vi "Test Launcher API.vi"() -> ()   [LabVIEW 2026]
doc: "Launcher API Tester."
uses:
  Mode.ctl
  ReplayMode.ctl
  RecordMode.ctl
  <vilib>/Utility/error.llb/DialogType.ctl
  Capture detection loop data--cluster.ctl
  663af669-4b40-4be5-87dd-68c6d9059199.vi
  <vilib>/Utility/error.llb/Search and Replace Pattern (string).vi
  <vilib>/JDP Science/JSONtext/Variant to JSON Text.vi
  <vilib>/JDP Science/JSONtext/LVClass Serializer/JSONtext LVClass Serializer.lvclass
  Launcher.lvlib
  replay/Replay/src/Libraries/Replay/Replay.lvlib
panel:
  in  "Load From Program Data":bool
  in  "key mode":enum16{"RELATIVE", "ABSOLUTE"}(ring)=enum."ABSOLUTE"
  in  "Load User Events":bool
  in  "Multicolumn Listbox":i32(listbox)
  in  "Run ID Replay":string="run-1791981803196"
  in  "Mode":T1={"Replay"=enum."None", "Record"=enum."User Events and Benchmarks"}
  out "last error":errorcluster
  in  "Show Diagram on Init":bool
  in  "Show Block Diagram":bool
  in  "Stop Module":bool
  in  "Start Module":bool
  in  "Hide Module Panel":bool
  in  "Show Module Panel":bool
  out "Status":string
  out "Module Running?":bool
  # "This VI tests the API for the Module."
  # "Set the folder where the runs are located\n\nCreate a loop or launch an asynchronous launcher that detects new runs\nOnce a new run is detected, launches the core module that polls the JSON files of the new run\nOnce the first frame is detected, cloneable module automatically launches a visualizer module."
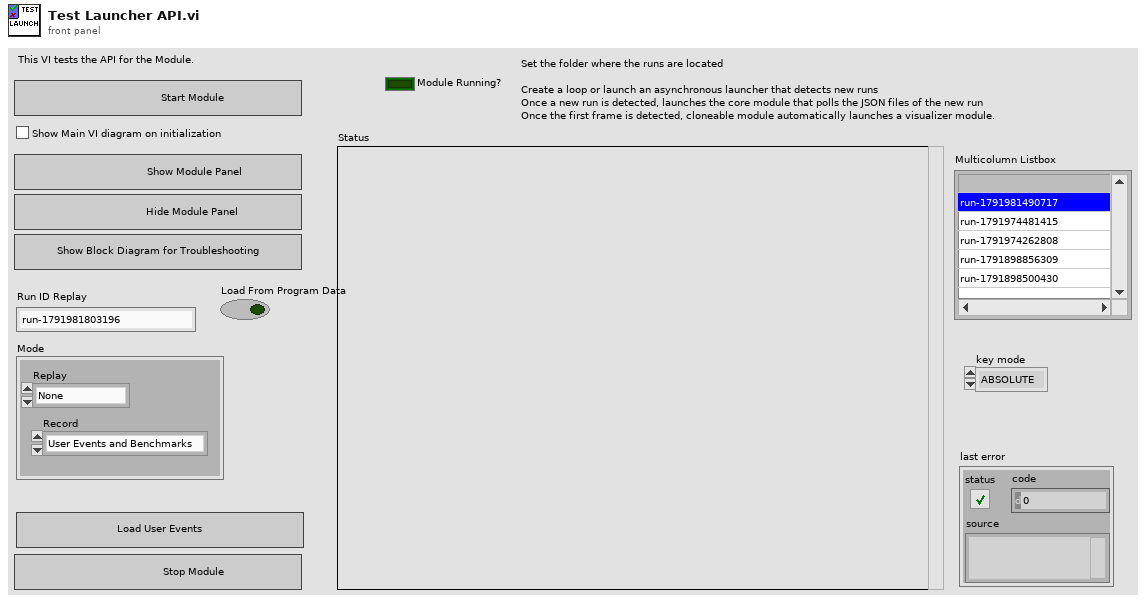
[diagram p1: front panel]
types:
  T1 = typedef "Mode.ctl" = cluster{"Replay":T2, "Record":T3}
  T2 = typedef "ReplayMode.ctl" = enum16{"None", "User Events"}
  T3 = typedef "RecordMode.ctl" = enum16{"None", "User Events", "Benchmarks", "User Events and Benchmarks"}
  T4 = typedef "Launcher.lvlib/Broadcast Events--cluster.ctl" = cluster{"Module Did Init":refnum<user-event>, "Status Updated":refnum<user-event>, "Error Reported":refnum<user-event>, "Module Did Stop":refnum<user-event>, "Update Module Execution Status":refnum<user-event>, "Start Capture Detection Loop":refnum<user-event>, "Benchmark Started":refnum<user-event>, "Broadcast number of frames and run ID":refnum<user-event>}
  T5 = typedef "DialogType.ctl" = u16
  T6 = typedef "Capture detection loop data--cluster.ctl" = cluster{"Period":i32, "Reset":bool, "Iteration":i32, "Capture":path, "Mode":T1, "Replay Run ID":string, "Frame Number":u32, "Core Module ID":i32, "EventRecorderLaunched":bool, "Frame 0 relative seconds":dbl, "Record Run ID":string}
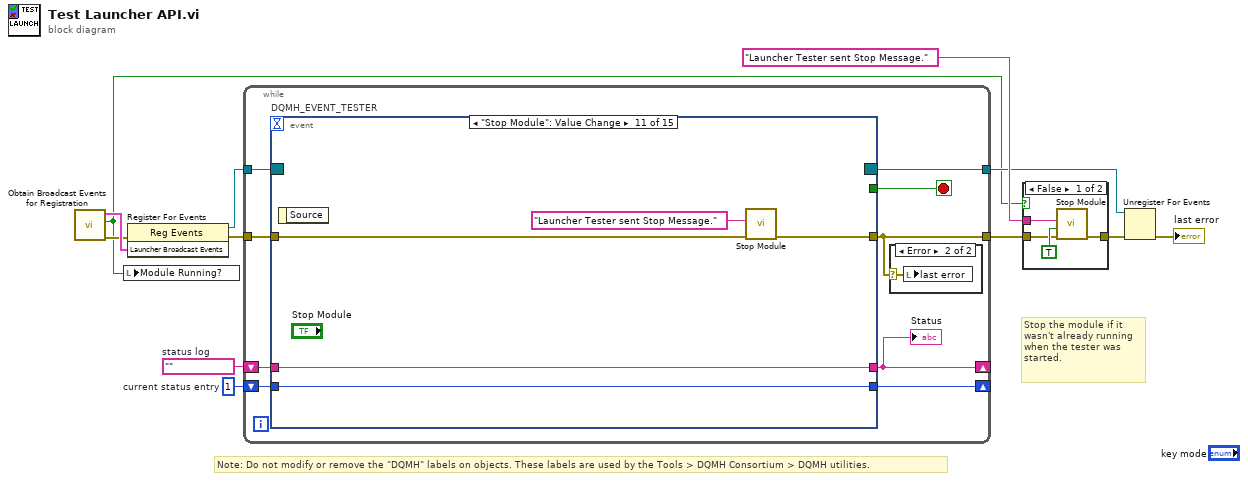
[diagram p0: block diagram]
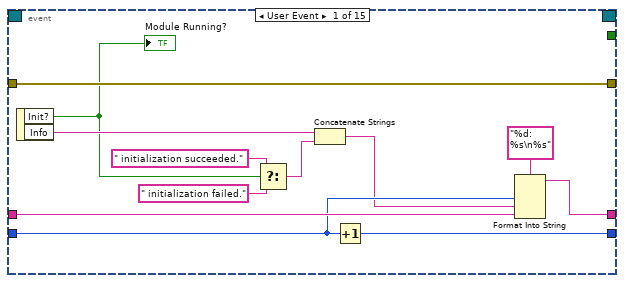
[diagram p4: hidden frame]
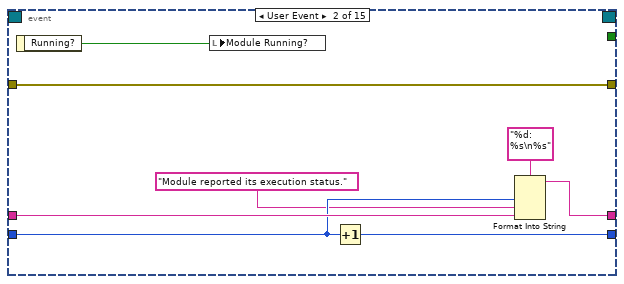
[diagram p5: hidden frame]
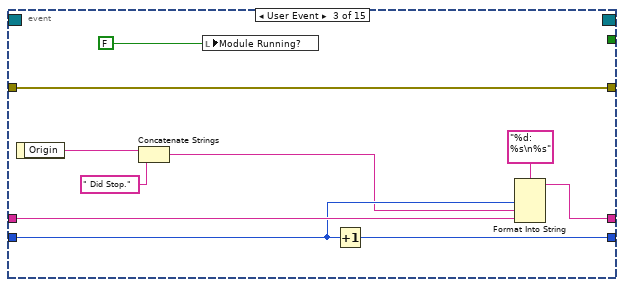
[diagram p6: hidden frame]
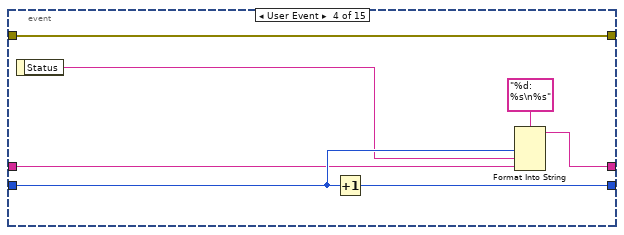
[diagram p7: hidden frame]
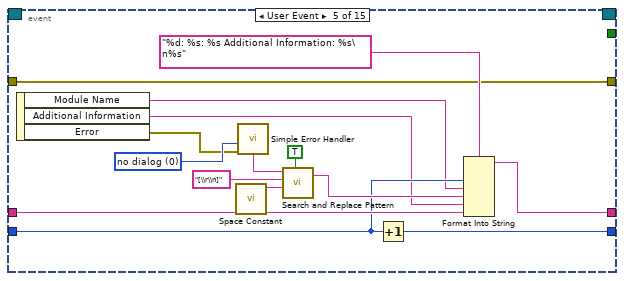
[diagram p8: hidden frame]
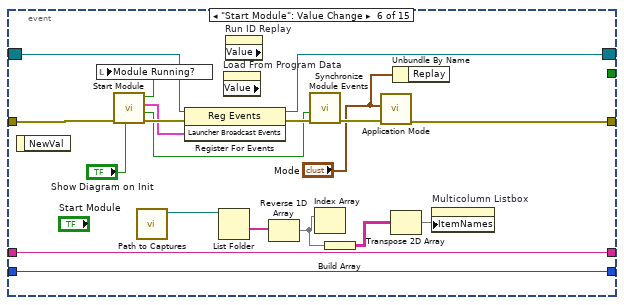
[diagram p9: hidden frame]
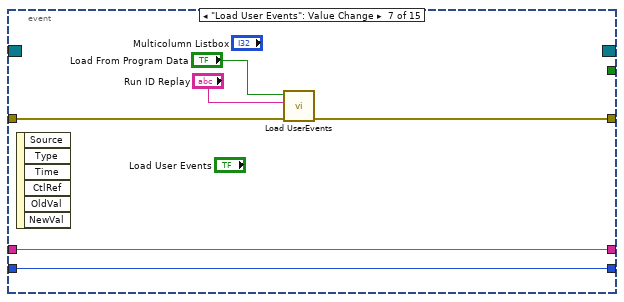
[diagram p10: hidden frame]
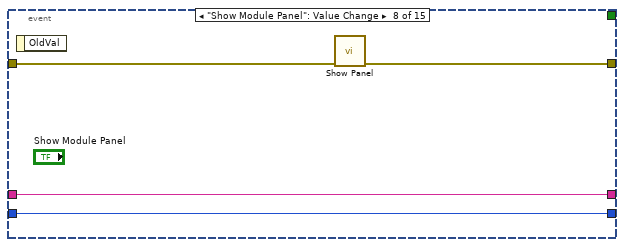
[diagram p11: hidden frame]
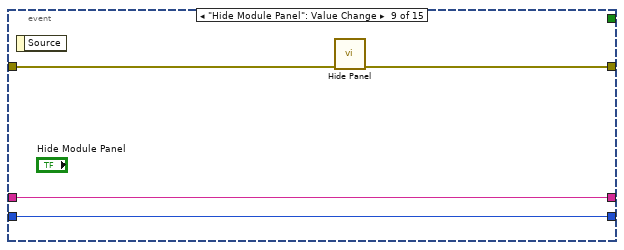
[diagram p12: hidden frame]
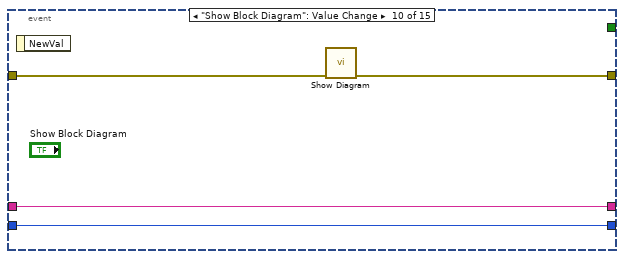
[diagram p13: hidden frame]
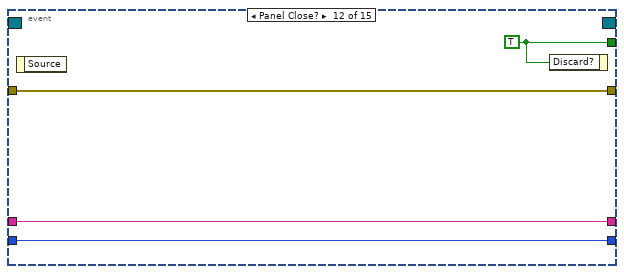
[diagram p14: hidden frame]
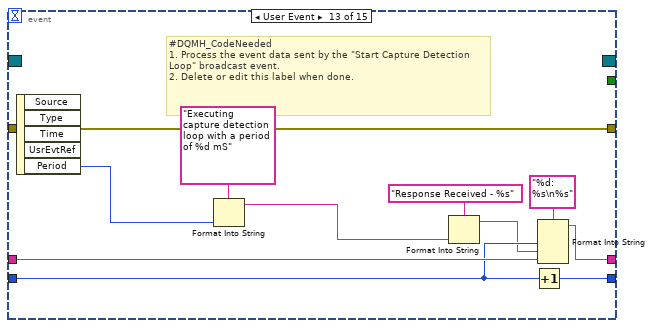
[diagram p15: hidden frame]
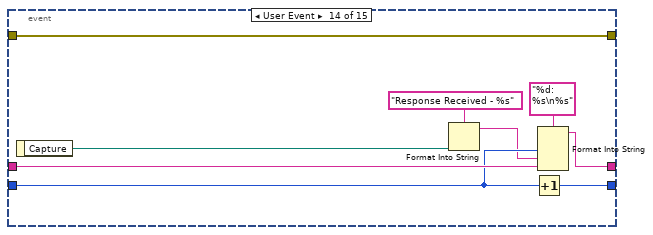
[diagram p16: hidden frame]
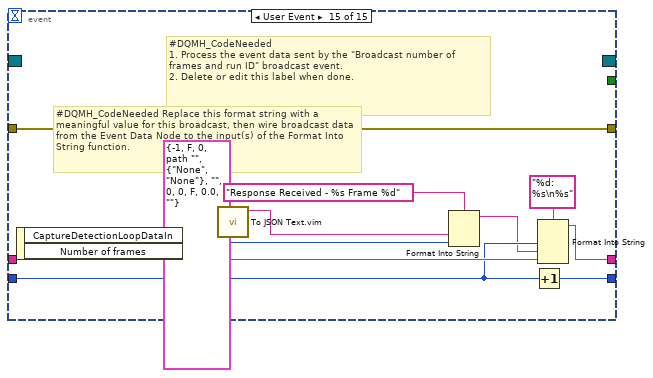
[diagram p17: hidden frame]
diagram:
  w9 = 1  # current status entry
  w10 = ""  # status log
  # "Stop the module if it wasn't already running when the tester was started."
  # "Note: Do not modify or remove the \"DQMH\" labels on objects. These labels are used by the Tools > DQMH Consortium > DQMH utilities."
  n1 = call "Obtain Broadcast Events for Registration.vi"() -> ("error out"=w4:errorcluster, "Already running?"=w3:bool, "Launcher Broadcast Events"=w7:T4)  [unwired: 9 in]
  n2 = local write "Module Running?"(w3) -> ()
  n3 = register-events(error in=w4, w7) -> (reference out=w6:refnum<event-registration>, error out=w8:errorcluster)  [unwired: 1 in]
  n4 = while {
    tunnel: w6 -> [w21]
    tunnel: [w13] -> w2
    shift-right: [w17] -> _
    shift-left: w10 -> [w19]
    shift-right: [w18] -> _
    shift-left: w9 -> [w20]
    tunnel: w8 -> [w16]
    tunnel: [w15] -> w5
    stop <- w14 stop-if-true
    n5 = event "DQMH_EVENT_TESTER" shown="[10] \"Stop Module\": Value Change" {
      selector: w21 -> [_ _ _ _ _ w87 _ _ _ _ _ _ _ _ _]
      dyn-events: [_ _ _ _ _ w86 _ _ _ _ _ _ _ _ _] -> w15
      timeout: _ -> [_ _ _ _ _ _ _ _ _ _ _ _ _ _ _]
      tunnel: [_ _ _ _ _ _ _ _ _ _ _ w120 _ _ _] -> w14
      tunnel: [w34 w36 w43 w53 w63 w76 w96 w103 w107 w108 w114 w117 w131 w140 w151] -> w13
      tunnel: w20 -> [w31 w40 w50 w56 w66 w90 w98 w101 w105 w109 w115 w118 w128 w137 w148]
      tunnel: w19 -> [w32 w41 w51 w55 w67 w91 w99 w102 w106 w110 w116 w119 w130 w139 w150]
      tunnel: [w29 w38 w48 w57 w65 w91 w99 w102 w106 w110 w116 w119 w129 w138 w149] -> w17
      tunnel: [w30 w39 w49 w59 w64 w90 w98 w101 w105 w109 w115 w118 w127 w136 w147] -> w18
      tunnel: w16 -> [w34 w36 w43 w53 w63 w85 w97 w100 w104 w111 w112 w117 w131 w140 w151]
      event User Event {
        n6 = event-data() -> ("Init?"=w26:bool, "Info"=w28:string)  [unwired: 1 in]
        "Module Running?" <- w26
        n7 = Select(t=" initialization succeeded.", s=w26, f=" initialization failed.") -> (s? t:f=w23:string)
        n8 = Concatenate Strings(w28, w23) -> (w27:string)
        n9 = Increment(x=w31) -> (x+1=w30:i32)
        n10 = Format Into String(format string="%d: %s\n%s", w31, w27, w32) -> (resulting string=w29:string)  [unwired: 2 in, 1 out]
      }
      event User Event {
        n11 = event-data() -> ("Running?"=w35:bool)  [unwired: 1 in]
        n12 = local write "Module Running?"(w35) -> ()
        n13 = Increment(x=w40) -> (x+1=w39:i32)
        n14 = Format Into String(format string="%d: %s\n%s", w40, "Module reported its execution status.", w41) -> (resulting string=w38:string)  [unwired: 2 in, 1 out]
      }
      event User Event {
        n15 = event-data() -> ("Origin"=w47:string)  [unwired: 1 in]
        n16 = Concatenate Strings(w47, " Did Stop.") -> (w46:string)
        n17 = local write "Module Running?"(FALSE ("Module Did Init?")) -> ()
        n18 = Increment(x=w50) -> (x+1=w49:i32)
        n19 = Format Into String(format string="%d: %s\n%s", w50, w46, w51) -> (resulting string=w48:string)  [unwired: 2 in, 1 out]
      }
      event User Event {
        n20 = event-data() -> ("Status"=w54:string)  [unwired: 1 in]
        n21 = Increment(x=w56) -> (x+1=w59:i32)
        n22 = Format Into String(format string="%d: %s\n%s", w56, w54, w55) -> (resulting string=w57:string)  [unwired: 2 in, 1 out]
      }
      event User Event {
        w68 = T5 0 items=["no dialog", "OK message", "continue or stop message", "OK message + warnings", "continue/stop + warnings"] ("type of dialog (OK msg:1)")
        n23 = event-data() -> ("Module Name"=w62:string, "Additional Information"=w61:string, "Error"=w60:errorcluster)  [unwired: 1 in]
        n24 = call <vilib>:"Space Constant.vi"() -> ("String"=w72:string)
        n25 = call <vilib>:"Simple Error Handler.vi"("type of dialog (OK msg:1)"=w68, "error in (no error)"=w60) -> ("message"=w69:string)  [unwired: 3 in, 4 out]
        n26 = call-poly <vilib>:"Search and Replace Pattern.vi"("string"=w69, "regular expression (\"\")"="[\\r\\n]" ("regular expression (\"\")"), "replace string (\"\")"=w72, "replace all? (F)"=TRUE ("replace all CR/LF with spaces")) -> ("result string"=w70:string)  [unwired: 1 in, 1 out]
        n27 = Increment(x=w66) -> (x+1=w64:i32)
        n28 = Format Into String(format string="%d: %s: %s Additional Information: %s\n%s", w66, w62, w70, w61, w67) -> (resulting string=w65:string)  [unwired: 2 in, 1 out]
      }
      event "Start Module": Value Change {
        n29 = event-data() -> ()  [unwired: 1 in, 1 out]
        n30 = call "Start Module.vi"("Show Main VI Diagram on Init (F)"="Show Diagram on Init", "error in"=w85) -> ("error out"=w92:errorcluster, "Wait for Event Sync?"=w89:bool, "Launcher Broadcast Events"=w88:T4, "Module Was Already Running?"=w84:bool)  [unwired: 5 in, 1 out]
        n31 = local write "Module Running?"(w84) -> ()
        n32 = call "Path to Captures.vi"() -> ("Captures"=w81:path)  [unwired: 11 in]
        n33 = register-events(reference=w87, error in=w92, w88) -> (reference out=w86:refnum<event-registration>, error out=w93:errorcluster)
        n34 = List Folder(path=w81) -> (folder names=w80:string[])  [unwired: 3 in, 3 out]
        n35 = property on="Load From Program Data" class="Bool (strict)" props=["Value"]() -> ()  [unwired: 2 in, 3 out]
        n36 = property on="Run ID Replay" class="Str" props=["Value"]() -> ()  [unwired: 2 in, 3 out]
        n37 = Reverse 1D Array(array=w80) -> (reversed array=w79:string[])
        n38 = call "Synchronize Module Events.vi"("error in"=w93, "Wait for Event Sync?"=w89) -> ("error out"=w82:errorcluster)  [unwired: 9 in]
        n39 = Index Array(array=w79) -> ()  [unwired: 1 in, 1 out]
        n40 = Build Array(w79) -> (w78:string[][])
        n41 = call "Application Mode.vi"("error in"=w82, "Mode"="Mode") -> ("error out"=w76:errorcluster)  [unwired: 9 in]
        n42 = Transpose 2D Array(2D array=w78) -> (transposed array=w77:string[][])
        n43 = Unbundle By Name("Mode") -> ()  [unwired: 1 out]
        n44 = property on="Multicolumn Listbox" class="MCListbox (strict)"("ItemNames"=w77) -> ()  [unwired: 2 in, 2 out]
      }
      event "Load User Events": Value Change {
        n45 = event-data() -> ()  [unwired: 1 in, 6 out]
        n46 = call "Load UserEvents.vi"("error in"=w97, "Run ID"="Run ID Replay", "Load From Program Data"="Load From Program Data") -> ("error out"=w96:errorcluster)  [unwired: 7 in, 1 out]
      }
      event "Show Module Panel": Value Change {
        n47 = event-data() -> ()  [unwired: 1 in, 1 out]
        n48 = call "Show Panel.vi"("error in"=w100) -> ("error out"=w103:errorcluster)  [unwired: 10 in]
      }
      event "Hide Module Panel": Value Change {
        n49 = event-data() -> ()  [unwired: 1 in, 1 out]
        n50 = call "Hide Panel.vi"("error in"=w104) -> ("error out"=w107:errorcluster)  [unwired: 10 in]
      }
      event "Show Block Diagram": Value Change {
        n51 = event-data() -> ()  [unwired: 1 in, 1 out]
        n52 = call "Show Diagram.vi"("error in"=w111) -> ("error out"=w108:errorcluster)  [unwired: 10 in]
      }
      event "Stop Module": Value Change {
        n53 = event-data() -> ()  [unwired: 1 in, 1 out]
        n54 = call "Stop Module.vi"("error in"=w112, "Origin"="Launcher Tester sent Stop Message.") -> ("error out"=w114:errorcluster)  [unwired: 9 in]
      }
      event Panel Close? {
        w120 = TRUE ("Discard?")
        n55 = event-data() -> ()  [unwired: 1 in, 1 out]
        n56 = event-data("Discard?"=w120) -> ()  [unwired: 1 in, 1 out]
      }
      event User Event {
        # "#DQMH_CodeNeeded\n1. Process the event data sent by the \"Start Capture Detection Loop\" broadcast event.\n2. Delete or edit this label when done."
        n57 = event-data() -> ("Period"=w122:i32)  [unwired: 1 in, 4 out]
        n58 = Format Into String(format string="Executing capture detection loop with a period of %d mS", w122) -> (resulting string=w121:string)  [unwired: 2 in, 1 out]
        n59 = Format Into String(format string="Response Received - %s", w121) -> (resulting string=w124:string)  [unwired: 2 in, 1 out]
        n60 = Increment(x=w128) -> (x+1=w127:i32)
        n61 = Format Into String(format string="%d: %s\n%s", w128, w124, w130) -> (resulting string=w129:string)  [unwired: 2 in, 1 out]
      }
      event User Event {
        n62 = event-data() -> ("Capture"=w132:path)  [unwired: 1 in]
        n63 = Format Into String(format string="Response Received - %s", w132) -> (resulting string=w133:string)  [unwired: 2 in, 1 out]
        n64 = Increment(x=w137) -> (x+1=w136:i32)
        n65 = Format Into String(format string="%d: %s\n%s", w137, w133, w139) -> (resulting string=w138:string)  [unwired: 2 in, 1 out]
      }
      event User Event {
        (unwired) T6 {"Period"=-1, "Reset"=FALSE, "Iteration"=0, "Capture"=path "", "Mode"={"Replay"=enum."None", "Record"=enum."None"}, "Replay Run ID"="", "Frame Number"=0, "Core Module ID"=0, "EventRecorderLaunched"=FALSE, "Frame 0 relative seconds"=0.0, "Record Run ID"=""} ("CaptureDetectionLoopDataIn")
        # "#DQMH_CodeNeeded Replace this format string with a meaningful value for this broadcast, then wire broadcast data from the Event Data Node to the input(s) of the Format Into String function."
        # "#DQMH_CodeNeeded\n1. Process the event data sent by the \"Broadcast number of frames and run ID\" broadcast event.\n2. Delete or edit this label when done."
        n66 = event-data() -> ("CaptureDetectionLoopDataIn"=w142:T6, "Number of frames"=w143:u32)  [unwired: 1 in]
        n67 = call "To JSON Text.vim"("Anything"=w142) -> ("<JSON>"=w141:string)  [unwired: 9 in, 1 out]
        n68 = Format Into String(format string="Response Received - %s Frame %d", w141, w143) -> (resulting string=w144:string)  [unwired: 2 in, 1 out]
        n69 = Increment(x=w148) -> (x+1=w147:i32)
        n70 = Format Into String(format string="%d: %s\n%s", w148, w144, w150) -> (resulting string=w149:string)  [unwired: 2 in, 1 out]
      }
    }
    "Status" <- w17
    n71 = case shown="Error" w13 {
      selector: w13 -> [_ w22]
      frame No Error {
      }
      frame Error {
        n72 = local write "last error"(w22) -> ()
      }
    }
  }
  n73 = case shown="False" w3 {
    tunnel: [w155 w156] -> w12
    tunnel: "Launcher Tester sent Stop Message." ("Origin") -> [w154 _]
    tunnel: w2 -> [w152 w156]
    frame False {
      n74 = call "Stop Module.vi"("error in"=w152, "Wait for Module to Stop? (F)"=TRUE ("Wait for Module to stop?"), "Origin"=w154) -> ("error out"=w155:errorcluster)  [unwired: 8 in]
    }
    frame True {
    }
  }
  n75 = Unregister For Events(event registration refnum=w5, error in=w12) -> (error out=→"last error":errorcluster)
